vi "W01_Packer.vi"() -> ()   [LabVIEW 2026]
doc: "Use this template to build a VI to use as a subVI."
panel:
  in  "quit":bool
  out "reject":bool
  out "grade":string
  out "running":bool
  out "why":string
  out "all OK":bool
  in  "stop machine":bool
  in  "start":bool
  in  "weight g":dbl
  in  "Auto mode":bool
  in  "Downstream ready":bool
  in  "Film loaded":bool
  in  "Seal temperature reached":bool
  in  "Air pressure OK":bool
  in  "E-stop released":bool
  in  "Door 2 closed":bool
  in  "Door 1 closed":bool
  # "Try: tick every condition except Film loaded, weight 503 -> Missing: Film loaded, Standard."
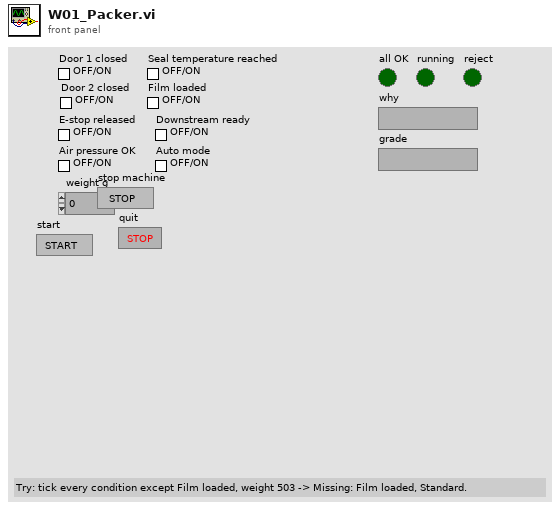
[diagram p1: front panel]
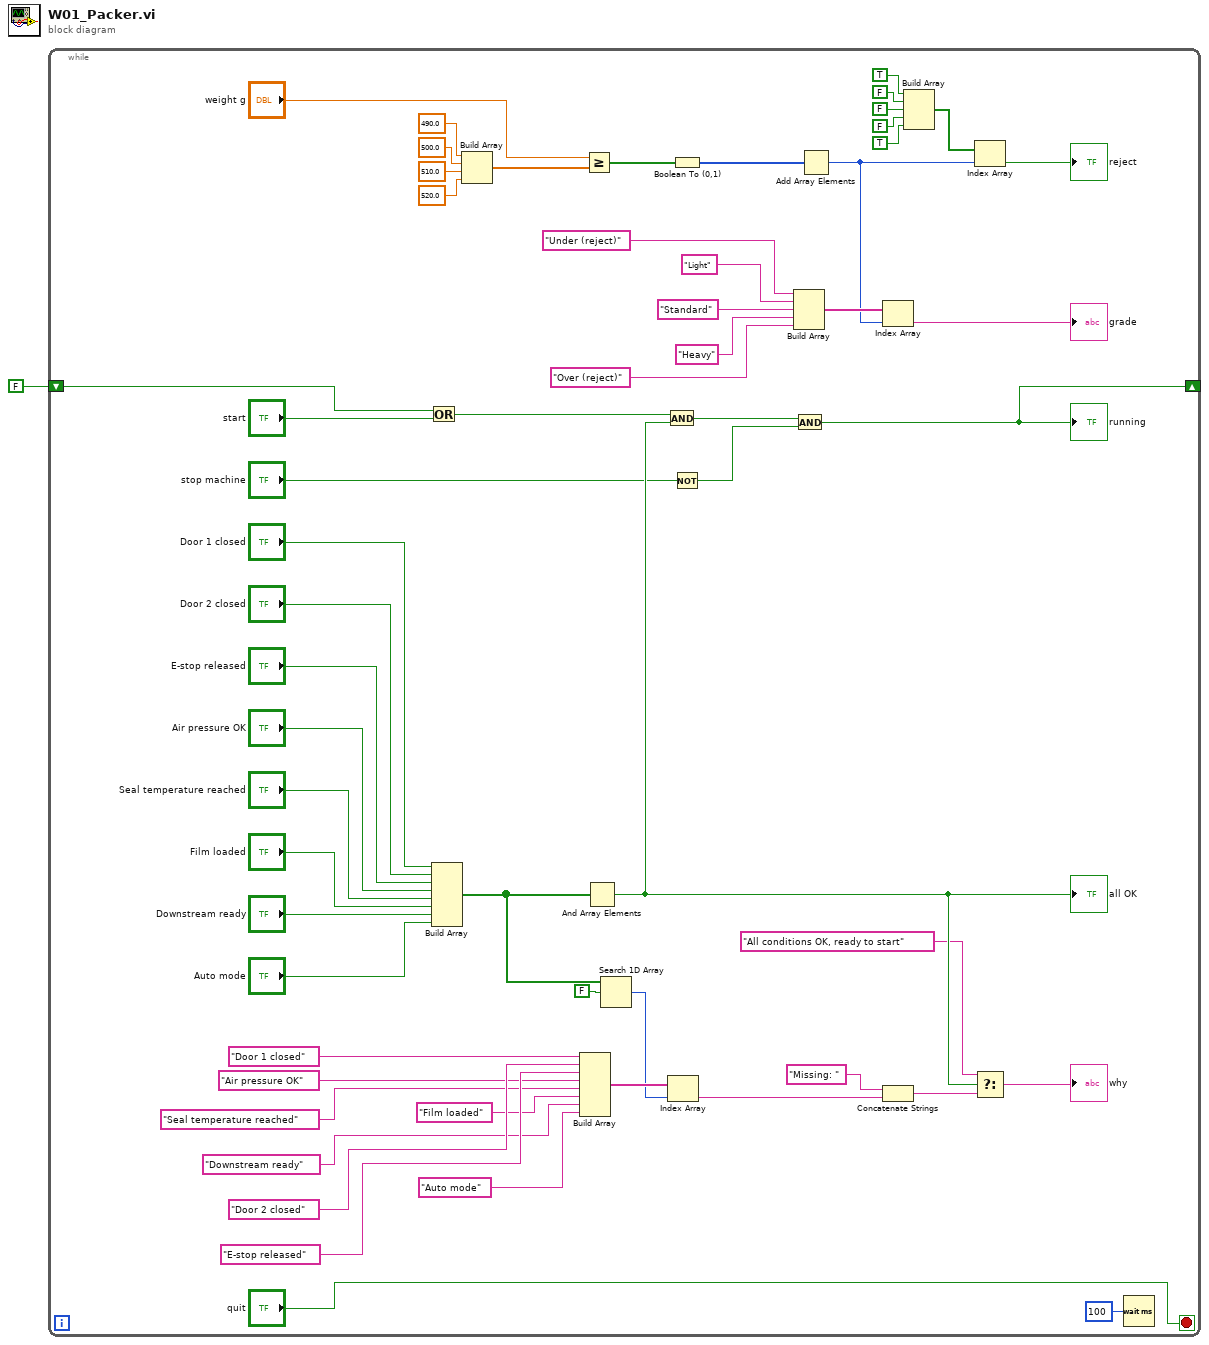
[diagram p0: block diagram]
diagram:
  n1 = while {
    shift-right: [w28] -> _
    shift-left: FALSE -> [w34]
    stop <- "quit" stop-if-true
    n2 = Or(x=w34, y="start") -> (x .or. y?=w32:bool)
    n3 = Build Array("Door 1 closed", "Door 2 closed", "E-stop released", "Air pressure OK", "Seal temperature reached", "Film loaded", "Downstream ready", "Auto mode") -> (w51:bool[])
    n4 = Build Array(490.0 ("x"), 500.0 ("x"), 510.0 ("x"), 520.0 ("x")) -> (w22:dbl[])
    n5 = Build Array("Door 1 closed", "Door 2 closed", "E-stop released", "Air pressure OK", "Seal temperature reached", "Film loaded", "Downstream ready", "Auto mode") -> (w41:string[])
    n6 = Greater Or Equal?(x="weight g", y=w22) -> (x >= y?=w21:bool[])
    n7 = And Array Elements(Boolean array=w51) -> (logical AND=w37:bool)
    "all OK" <- w37
    n8 = Search 1D Array(1D array=w51, element=FALSE) -> (index of element=w40:i32)  [unwired: 1 in]
    n9 = And(x=w32, y=w37) -> (x .and. y?=w30:bool)
    n10 = Index Array(array=w41, index=w40) -> (element=w38:string)
    n11 = Boolean To (0,1)(Boolean=w21) -> (0, 1=w20:i16[])
    n12 = Not(x="stop machine") -> (.not. x?=w29:bool)
    n13 = Build Array("Under (reject)", "Light", "Standard", "Heavy", "Over (reject)") -> (w14:string[])
    n14 = And(x=w30, y=w29) -> (x .and. y?=w28:bool)
    "running" <- w28
    n15 = Add Array Elements(numeric array=w20) -> (sum=w13:i16)
    n16 = Index Array(array=w14, index=w13) -> (element=→"grade":string)
    n17 = Concatenate Strings("Missing: ", w38) -> (w35:string)
    n18 = Build Array(TRUE, FALSE, FALSE, FALSE, TRUE) -> (w7:bool[])
    n19 = Index Array(array=w7, index=w13) -> (element=→"reject":bool)
    n20 = Select(t="All conditions OK, ready to start", s=w37, f=w35) -> (s? t:f=→"why":string)
    n21 = Wait (ms)(milliseconds to wait=u32 100) -> ()  [unwired: 1 out]
  }
